vi "RT_ShVariables.vi"() -> ()   [LabVIEW 2025]
panel:
  out "error IO":errorcluster
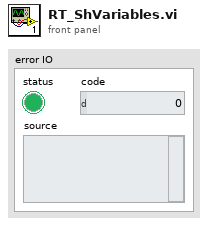
[diagram p1: front panel]
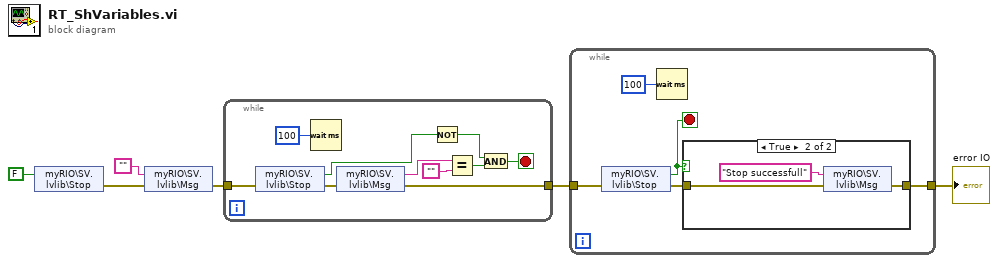
[diagram p0: block diagram]
diagram:
  n1 = shared-variable "myRIO\\SV.lvlib\\Stop"(FALSE ("Stop")) -> (error out=w6:errorcluster)  [unwired: 1 in]
  n2 = shared-variable "myRIO\\SV.lvlib\\Msg"("", error in=w6) -> (error out=w4:errorcluster)
  n3 = while {
    tunnel: w4 -> [w15]
    tunnel: [w10] -> w2
    stop <- w7 stop-if-true
    n4 = shared-variable "myRIO\\SV.lvlib\\Stop"(error in=w15) -> (w14:bool, error out=w16:errorcluster)
    n5 = Wait (ms)(milliseconds to wait=u32 100) -> ()  [unwired: 1 out]
    n6 = shared-variable "myRIO\\SV.lvlib\\Msg"(error in=w16) -> (w12:string, error out=w10:errorcluster)
    n7 = Not(x=w14) -> (.not. x?=w13:bool)
    n8 = Equal?(x=w12, y="") -> (x = y?=w9:bool)
    n9 = And(x=w13, y=w9) -> (x .and. y?=w7:bool)
  }
  n10 = while {
    tunnel: w2 -> [w21]
    tunnel: [w19] -> w1
    stop <- w18 stop-if-true
    n11 = shared-variable "myRIO\\SV.lvlib\\Stop"(error in=w21) -> (w18:bool, error out=w20:errorcluster)
    n12 = Wait (ms)(milliseconds to wait=u32 100) -> ()  [unwired: 1 out]
    n13 = case shown="True" w18 {
      tunnel: w20 -> [w22 w25]
      tunnel: [w22 w23] -> w19
      frame False {
      }
      frame True {
        n14 = shared-variable "myRIO\\SV.lvlib\\Msg"("Stop successfull" ("Msg"), error in=w25) -> (error out=w23:errorcluster)
      }
    }
  }
  "error IO" <- w1
